vi "Dispatch Probe.vi"() -> (0 "answer":string)   [LabVIEW 2026]
doc: "Round15 P15: calls Sensor:Tag through a dynamic-dispatch terminal. The diagram constant 'seed' is a path stand-in that lvai_swap_subvis constantsJson turns into a class constant; which class it names decides which implementation runs. answer=Temp Sensor proves dynamic dispatch; answer=Sensor proves it does not."
uses:
  lib/Sensor.lvclass
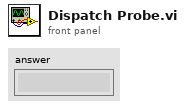
[diagram p1: front panel]
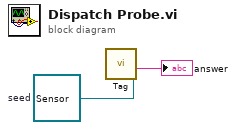
[diagram p0: block diagram]
diagram:
  w1 = refnum<class "Sensor.lvclass"> refnum  # seed
  n1 = call-dynamic "Tag.vi"("obj in"=w1) -> ("tag"=→"answer":string)  [unwired: 10 in]
